vi "Reset (no conIdx, never a member).vi"() -> ()   [LabVIEW 2026]
doc: "Round14 A/B: identical in shape to Sensor's override but with NO conIdx on any terminal. Asked one question - does lvai_add_class_method's panePattern step (4815) put terminals on the pane by itself, or is conIdx the only thing that ever does (round 13's LV014)?"
panel:
  out "obj out":path
  in  "obj in":path
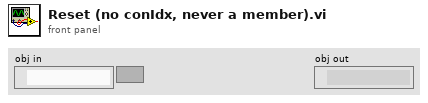
[diagram p1: front panel]
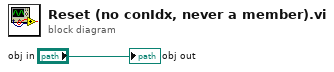
[diagram p0: block diagram]
diagram:
  "obj out" <- "obj in"
